vi "Indexed History.vi"(10 "seconds":i32=600, 11 "price history":dbl[][](array[numeric])) -> (3 "indexed history":dbl[][](array[numeric]))   [LabVIEW 2020, in "Full Featured MCP Server.lvlib"]
doc: "Prepares the price history for one chart of all stocks: the last seconds of every stock, scaled so each curve starts at 100. Stocks of 10 and of 400 euros become comparable, and a trend shows as a curve leaving 100."
uses:
  Full Featured MCP Server.lvlib
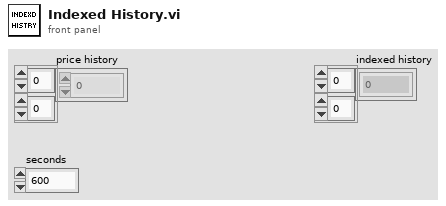
[diagram p1: front panel]
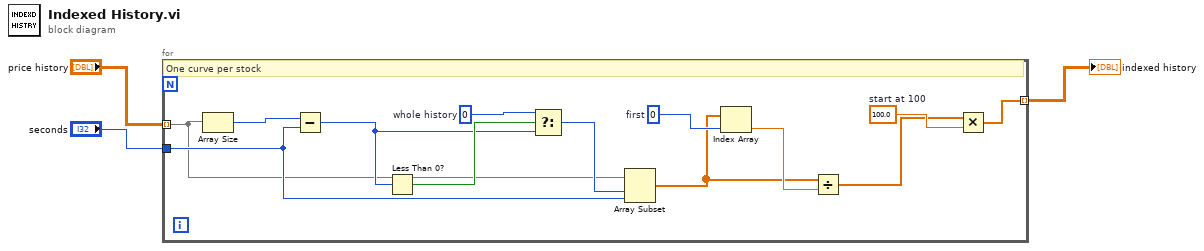
[diagram p0: block diagram]
diagram:
  n1 = for {
    tunnel: "price history" -> [w4] mode=indexing
    tunnel: "seconds" -> [w6]
    tunnel: [w16] -> w3 mode=indexing
    w15 = 100.0  # start at 100
    w12 = 0  # first
    w9 = 0  # whole history
    # "One curve per stock"
    n2 = Array Size(array=w4) -> (size(s)=w5:i32)
    n3 = Subtract(x=w5, y=w6) -> (x-y=w7:i32)
    n4 = Less Than 0?(x=w7) -> (x < 0?=w8:bool)
    n5 = Select(t=w9, s=w8, f=w7) -> (s? t:f=w10:i32)
    n6 = Array Subset(array=w4, index=w10, length=w6) -> (w11:dbl[])
    n7 = Index Array(array=w11, index=w12) -> (element=w13:dbl)
    n8 = Divide(x=w11, y=w13) -> (x/y=w14:dbl[])
    n9 = Multiply(x=w14, y=w15) -> (x*y=w16:dbl[])
  }
  "indexed history" <- w3
